vi "close.vi"(8 "error in (no error)":errorcluster, 11 "PackageFile in":refnum<class "PackageFile.lvclass">) -> (0 "error out":errorcluster, 3 "path":path)   [LabVIEW 2020, in "vi_package_building_extensions.lvlib" / "PackageFile.lvclass"]
uses:
  PackageFile.lvclass
  PackageFile.lvclass/PackageFile.ctl
  vi_package_building_extensions.lvlib
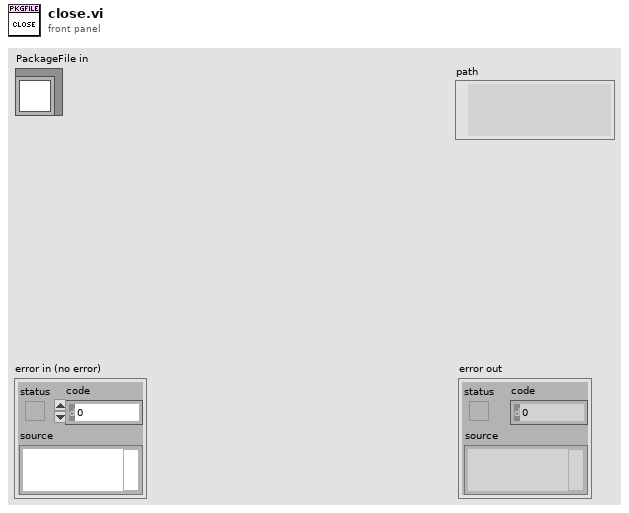
[diagram p1: front panel]
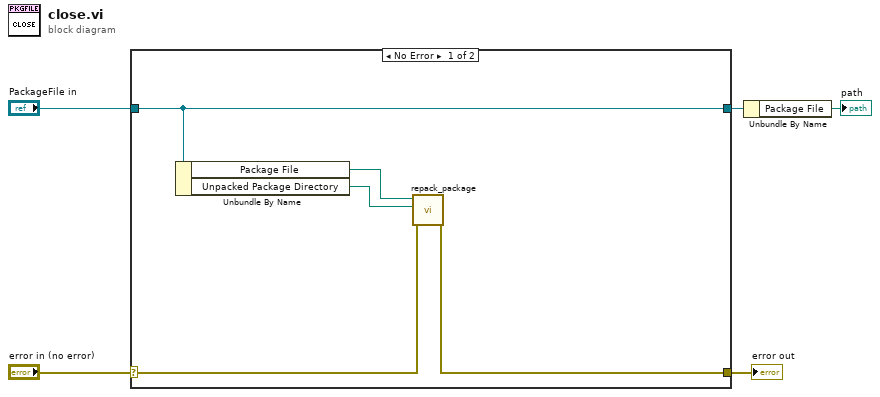
[diagram p0: block diagram]
diagram:
  n1 = case shown="No Error" "error in (no error)" {
    selector: "error in (no error)" -> [w7 w12]
    tunnel: [w6 w12] -> w4
    tunnel: [w10 w11] -> w2
    tunnel: "PackageFile in" -> [w10 w11]
    frame No Error {
      n2 = Unbundle By Name(w10) -> ("Package File"=w9:path, "Unpacked Package Directory"=w8:path)
      n3 = call "repack_package.vi"("error in (no error)"=w7, "Unpacked Package Directory"=w8, "Package File"=w9) -> ("error out"=w6:errorcluster)  [unwired: 8 in]
    }
    frame Error {
    }
  }
  "error out" <- w4
  n4 = Unbundle By Name(w2) -> ("Package File"=→"path":path)
